vi "Import from Project.vi"(8 "error in":errorcluster, 11 "references":T1) -> (0 "error out":errorcluster, 3 "references out":T1)   [LabVIEW 2015, in "Scan Engine editor node.lvclass"]
uses:
  Scan Engine editor node.lvclass
  <vilib>/NI/DCAF/Tag Editor Core/Table API/Table Manager/object ref.ctl
  <vilib>/NI/DCAF/Tag Editor Core/Configuration Editor/Classes/Engine Parent/Engine Parent Editor Node.lvclass
  <vilib>/NI/DCAF/Tag Editor Core/Configuration Editor/Classes/Module editor node/module editor node.lvclass
  configuration/Scan Engine configuration.lvclass
  <vilib>/NI/DCAF/Tag Editor Core/Configuration Editor/Classes/Module editor node/Read Module Configuration.vi
  <vilib>/NI/DCAF/Tag Editor Core/Configuration Editor/Classes/Module editor node/Write Module Configuration.vi
  <vilib>/NI/Tag Bus Module Framework/module configuration/TBM module configuration.lvclass
  <vilib>/NI/DCAF/Tag Editor Core/Table API/Table Manager/Table Manager.lvclass
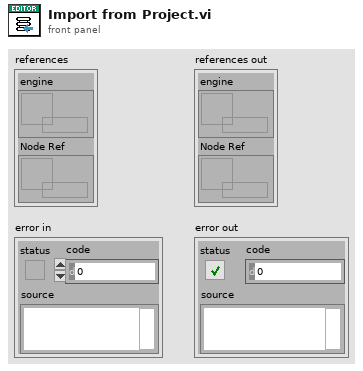
[diagram p1: front panel]
types:
  T1 = typedef "Table Manager.lvlib/Table Manager.lvclass/object ref.ctl" = cluster{"engine":refnum<data-value>, "Node Ref":refnum<data-value>}
  T2 = typedef "Scan Engine configuration.lvclass/Line.ctl" = cluster{"channel":refnum<class "TBM channel.lvclass">, "Tag":string}
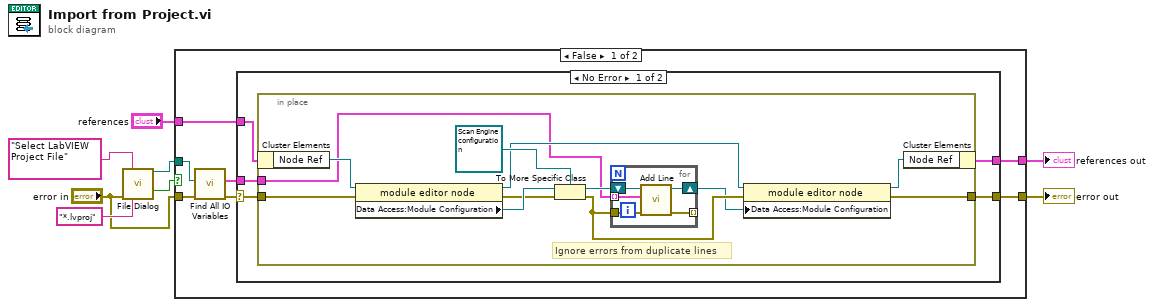
[diagram p0: block diagram]
diagram:
  n1 = call "File Dialog"("prompt"="Select LabVIEW Project File", "error in"="error in", "pattern (all files)"="*.lvproj") -> ("selected path"=w6:path, "cancelled"=w2:bool)  [unwired: 9 in, 2 out]
  n2 = case shown="False" w2 {
    tunnel: w6 -> [w15 _]
    tunnel: "references" -> [w13 w41]
    tunnel: [w11 w41] -> w4
    tunnel: [w10 w40] -> w3
    tunnel: "error in" -> [w9 w40]
    frame False {
      n3 = call "Find All IO Variables.vi"("error in"=w9, "Path"=w15) -> ("error out"=w14:errorcluster, "Tags"=w12:T2[])  [unwired: 8 in]
      n4 = case shown="No Error" w14 {
        selector: w14 -> [w18 w38]
        tunnel: w13 -> [w20 w39]
        tunnel: w12 -> [w19 _]
        tunnel: [w17 w39] -> w11
        tunnel: [w16 w38] -> w10
        frame No Error {
          n5 = in-place {
            in-place-border: w19 -> [w21]
            in-place-border: w18 -> [w29]
            in-place-border: [w25] -> w16
            # "Ignore errors from duplicate lines"
            n6 = in-place-cluster #1(w20) -> ("Node Ref"=w32:refnum<data-value>)
            n7 = property class="module editor node"(reference=w32, error in=w29) -> (reference out=w28:refnum<data-value>, error out=w27:errorcluster, "Data Access:Module Configuration"=w30:refnum<class "TBM module configuration.lvclass">)
            n8 = To More Specific Class(target class=refnum<class "Scan Engine configuration.lvclass"> refnum ("Scan Engine configuration"), reference=w30, error in=w27) -> (specific class reference=w24:refnum<class "Scan Engine configuration.lvclass">, error out=w23:errorcluster)
            n9 = for {
              tunnel: w23 -> [w36]
              shift-right: [w35] -> w22
              shift-left: w24 -> [w37]
              tunnel: [w34] -> _ mode=indexing
              tunnel: w21 -> [w33] mode=indexing
              n10 = call "Add Line.vi"("error in"=w36, "Line"=w33, "Scan Engine configuration in"=w37) -> ("error out"=w34:errorcluster, "Scan Engine configuration out"=w35:refnum<class "Scan Engine configuration.lvclass">)  [unwired: 7 in]
            }
            n11 = property class="module editor node"(reference=w28, error in=w23, "Data Access:Module Configuration"=w22) -> (reference out=w26:refnum<data-value>, error out=w25:errorcluster)
            n12 = in-place-cluster #1("Node Ref"=w26) -> (w17:T1)
          }
        }
        frame Error {
        }
      }
    }
    frame True {
    }
  }
  "references out" <- w4
  "error out" <- w3
